vi "BioMapWriteCore.vi"(6 "conv. coeff.":sgl=655.0, 7 "Image in":dbl[][][](array[numeric]), 8 "error in":errorcluster, 9 "Y_img":i32, 10 "Image Params":T1={"File Header"={"Start Position"=[], "StepWidth"=[0.05, 0.05], "Dimension"=[], "SpecLength"=10000}, "mzCali."=[0.0, 1.0, 0.0], "m/z_Array"=[0.0, 1.0, 0.0], "SampleRate"=0.0, "TrigDelay"=0.0, "file refnum"=refnum, "file path"=path "", "PeakOI"=[], "Binning"={"Enable"=FALSE, "BinType"=enum."ByScreen", "BinWidth"=0.5, "Maximum"=0.0, "Minimum"=0.0}} {"SampleRate" items=["50MS/s"=50000000.0, "100MS/s"=100000000.0, "125MS/s"=125000000.0, "200MS/s"=200000000.0, "250MS/s"=250000000.0, "500MS/s"=500000000.0, "1GS/s"=1000000000.0, "1.6GS/s"=1600000000.0]}, 11 "data buffer in":refnum<queue>) -> (0 "error out":errorcluster, 2 "file refnum out":refnum<file>, 5 "Image out":dbl[][][](array[numeric]))   [LabVIEW 2013]
uses:
  BioMAPWriterCoreParams.ctl
  Files/BinaryHeader.ctl
  ControlDef/SampleRateSelector.ctl
  Binning/BinType.ctl
panel:
  out "#element":i32
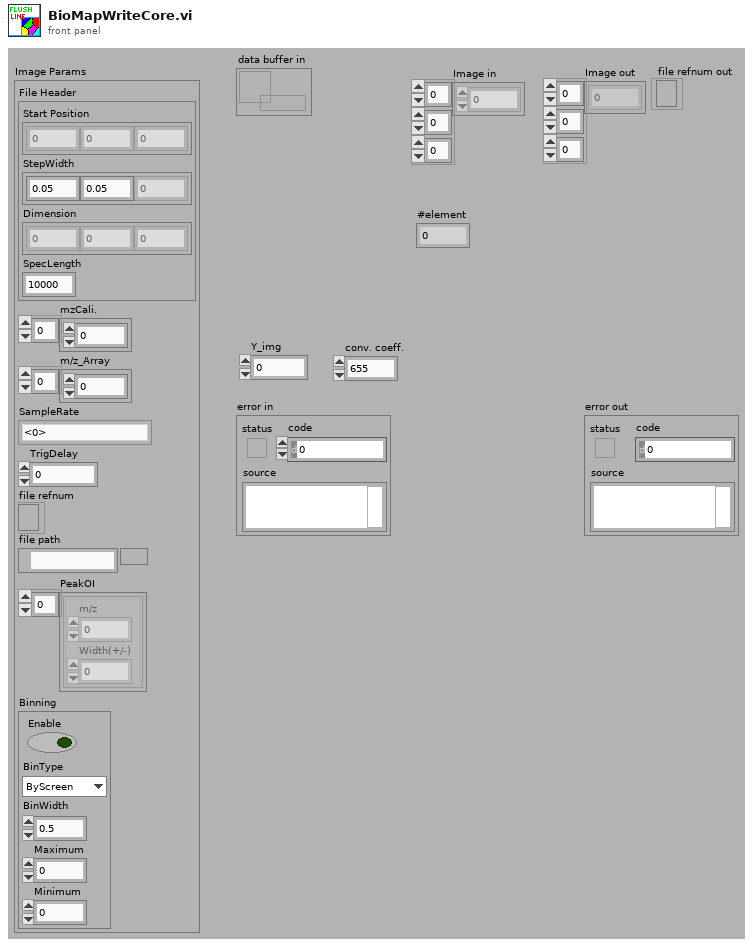
[diagram p1: front panel]
types:
  T1 = typedef "BioMAPWriterCoreParams.ctl" = cluster{"File Header":T2, "mzCali.":dbl[], "m/z_Array":dbl[], "SampleRate":T3, "TrigDelay":dbl, "file refnum":refnum<file>, "file path":path, "PeakOI":cluster{"m/z":dbl, "Width(+/-)":dbl}[], "Binning":cluster{"Enable":bool, "BinType":T4, "BinWidth":dbl, "Maximum":dbl, "Minimum":dbl}}
  T2 = typedef "BinaryHeader.ctl" = cluster{"Start Position":dbl[], "StepWidth":dbl[], "Dimension":i32[], "SpecLength":i32}
  T3 = typedef "SampleRateSelector.ctl" = dbl
  T4 = typedef "BinType.ctl" = enum16{"ByTime", "ByScreen", "ByMass", "ToUnitMass"}
  T5 = enum16{"big-endian, network order", "native, host order", "little-endian"}
  T6 = cluster{"Average":i32, "X (Img)":i32, "Y (Img)":i32, "Spectra":sgl[]}[]
  T7 = cluster{"Average":i32, "X (Img)":i32, "Y (Img)":i32, "Spectra":sgl[]}
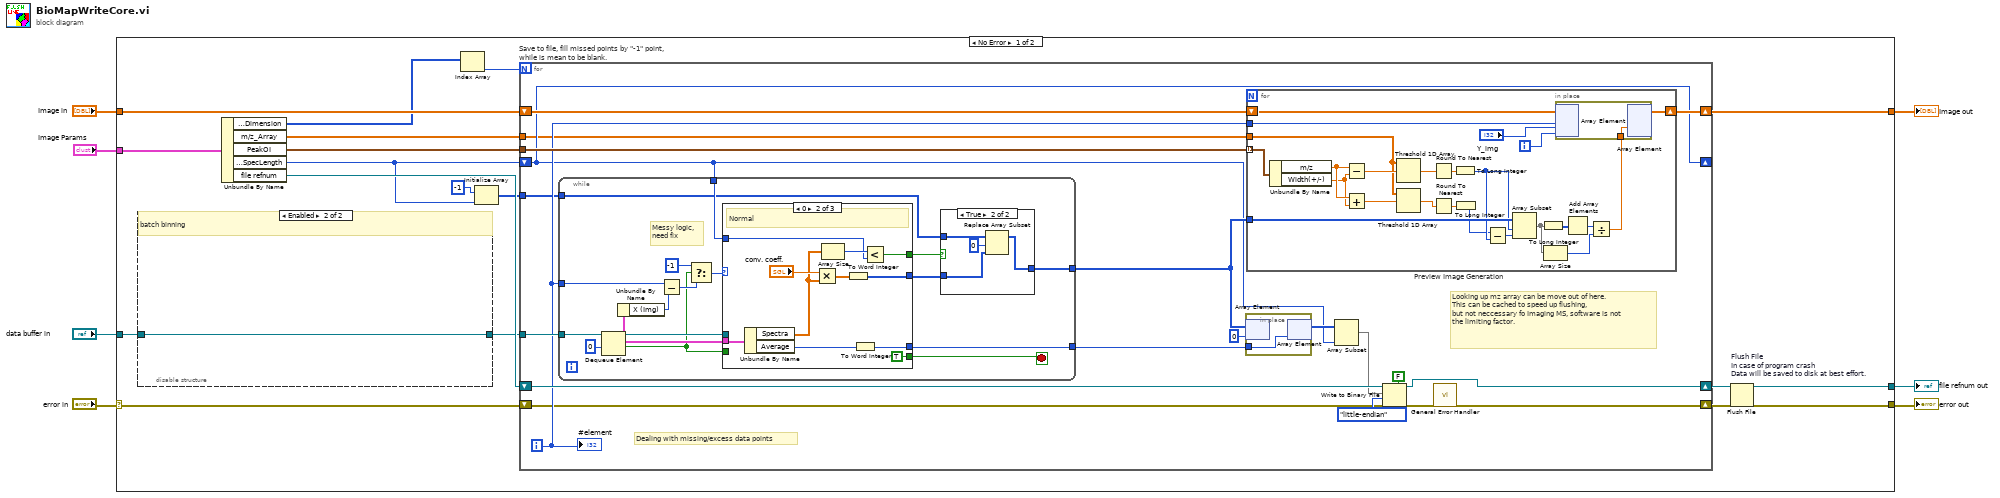
[diagram p0: block diagram]
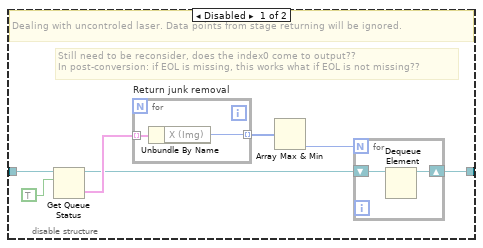
[diagram p2: hidden frame]
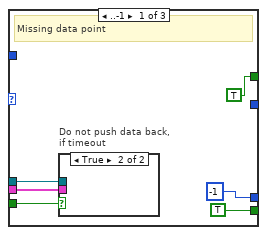
[diagram p4: hidden frame]
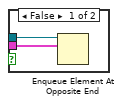
[diagram p5: hidden frame]
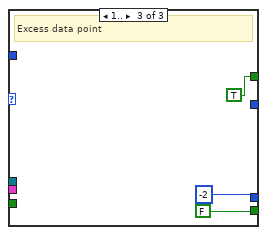
[diagram p6: hidden frame]
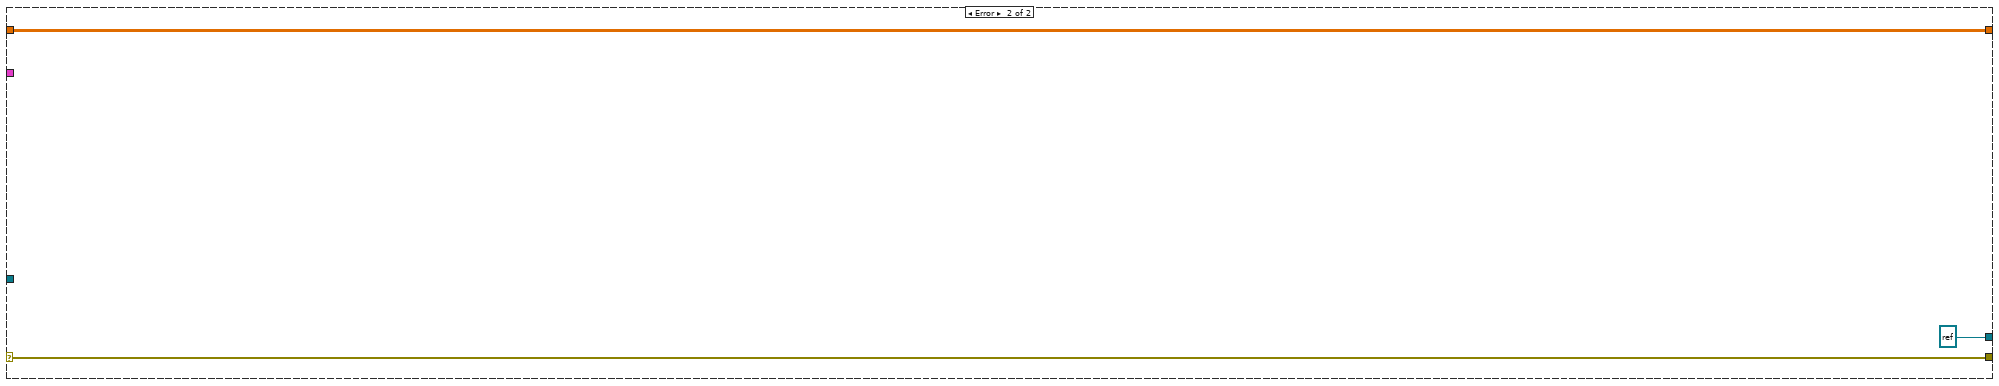
[diagram p7: hidden frame]
diagram:
  n1 = case shown="No Error" "error in" {
    selector: "error in" -> [w22 w130]
    tunnel: [w25 w128] -> w7
    tunnel: [w12 w130] -> w6
    tunnel: [w14 refnum<file> refnum ("file refnum")] -> w5
    tunnel: "Image in" -> [w23 w128]
    tunnel: "data buffer in" -> [w11 _]
    tunnel: "Image Params" -> [w9 _]
    frame No Error {
      n2 = disable-structure shown="Enabled" {
        disable-tunnel: w11 -> [w30 w37]
        disable-tunnel: [w28 w37] -> w17
        frame Disabled {
          # "Still need to be reconsider, does the index0 come to output??\nIn post-conversion: if EOL is missing, this works what if EOL is not missing??"
          # "Dealing with uncontroled laser. Data points from stage returning will be ignored."
          n3 = Get Queue Status(queue=w30, return elements? (F)=TRUE) -> (queue out=w29:refnum<queue>, elements=w32:T6)  [unwired: 1 in, 6 out]
          n4 = for "Return junk removal" {
            tunnel: w32 -> [w36] mode=indexing
            tunnel: [w35] -> w27 mode=indexing
            n5 = Unbundle By Name(w36) -> ("X (Img)"=w35:i32)
          }
          n6 = Array Max & Min(array=w27) -> (min index (indices)=w26:i32)  [unwired: 3 out]
          n7 = for {
            N: w26 -> [_]
            shift-right: [w33] -> w28
            shift-left: w29 -> [w34]
            n8 = Dequeue Element(queue=w34) -> (queue out=w33:refnum<queue>)  [unwired: 2 in, 3 out]
          }
        }
        frame Enabled {
          # "batch binning"
        }
      }
      n9 = Unbundle By Name(w9) -> ("File Header.Dimension"=w21:i32[], "m/z_Array"=w8:dbl[], "PeakOI"=w19:cluster{"m/z":dbl, "Width(+/-)":dbl}[], "File Header.SpecLength"=w10:i32, "file refnum"=w20:refnum<file>)
      n10 = Index Array(array=w21) -> (element=w18:i32)  [unwired: 1 in]
      n11 = Initialize Array(i16 -1 ("element"), w10) -> (w15:i16[])
      n12 = for "Save to file, fill missed points by \"-1\" point, while is mean to be blank." {
        N: w18 -> [_]
        shift-right: [w51] -> w13
        shift-left: w22 -> [w40]
        shift-right: [w54] -> w25
        shift-left: w23 -> [w53]
        tunnel: w17 -> [w57]
        shift-right: [w55] -> w24
        shift-left: w20 -> [w56]
        tunnel: w19 -> [w52]
        tunnel: w8 -> [w38]
        tunnel: w15 -> [w41]
        shift-right: [w39] -> _
        shift-left: w10 -> [w39]
        i -> [w42]
        # "Looking up mz array can be move out of here.\nThis can be cached to speed up flushing, \nbut not neccessary fo Imaging MS, software is not \nthe limiting factor."
        # "Dealing with missing/excess data points"
        n13 = while {
          tunnel: w57 -> [w74]
          tunnel: [w68] -> w44
          tunnel: w39 -> [w67]
          tunnel: [w62] -> w43
          tunnel: w42 -> [w63]
          tunnel: w41 -> [w60]
          stop <- w66 stop-if-true
          # "Messy logic,\nneed fix"
          n14 = Dequeue Element(queue=w74, timeout in ms (-1)=0) -> (queue out=w70:refnum<queue>, element=w69:T7, timed out?=w59:bool)  [unwired: 1 in, 1 out]
          n15 = Unbundle By Name(w69) -> ("X (Img)"=w72:i32)
          n16 = Subtract(x=w63, y=w72) -> (x-y=w71:i32)
          n17 = Select(t=-1, s=w59, f=w71) -> (s? t:f=w65:i32)
          n18 = case shown="0" w65 {
            tunnel: w70 -> [w82 _ _]
            tunnel: w69 -> [w81 w98 _]
            tunnel: [i16 -1 ("Average") w96 i16 -2 ("Average")] -> w68
            tunnel: w67 -> [_ w91 _]
            tunnel: [TRUE TRUE FALSE] -> w66
            tunnel: [_ w90 _] -> w61
            tunnel: [TRUE w89 TRUE] -> w58
            tunnel: w59 -> [w80 _ _]
            frame ..-1 {
              # "Missing data point"
              n19 = case "Do not push data back, \nif timeout" shown="True" w80 {
                tunnel: w82 -> [w87 _]
                tunnel: w81 -> [w86 _]
                frame False {
                  n20 = Enqueue Element At Opposite End(queue=w87, element=w86) -> ()  [unwired: 2 in, 3 out]
                }
                frame True {
                }
              }
            }
            frame 0 {
              # "Normal"
              n21 = Unbundle By Name(w98) -> ("Spectra"=w88:sgl[], "Average"=w95:i32)
              n22 = Multiply(x="conv. coeff.", y=w88) -> (x*y=w97:sgl[])
              n23 = Array Size(array=w88) -> (size(s)=w92:i32)
              n24 = To Word Integer(number=w97) -> (16bit integer=w90:i16[])
              n25 = To Word Integer(number=w95) -> (16bit integer=w96:i16)
              n26 = Less?(x=w92, y=w91) -> (x < y?=w89:bool)
            }
            frame 1.. {
              # "Excess data point"
            }
          }
          n27 = case shown="True" w58 {
            tunnel: [w75 w79] -> w62
            tunnel: w61 -> [w75 w77]
            tunnel: w60 -> [_ w78]
            frame False {
            }
            frame True {
              n28 = Replace Array Subset(array=w78, new element=w77, index=0) -> (w79:i16[])
            }
          }
        }
        n29 = in-place {
          in-place-border: w44 -> [w127]
          n30 = in-place-array #1(w43, 0) -> ()  [unwired: 1 out]
          n31 = in-place-array #1(w127) -> (w45:i16[])  [unwired: 1 out]
        }
        n32 = for "Preview Image Generation" {
          shift-right: [w112] -> w54
          shift-left: w53 -> [w119]
          tunnel: w52 -> [w125] mode=indexing
          tunnel: w43 -> [w118]
          tunnel: w38 -> [w121]
          tunnel: w42 -> [w105]
          i -> [w104]
          n33 = Unbundle By Name(w125) -> ("m/z"=w124:dbl, "Width(+/-)"=w123:dbl)
          n34 = Subtract(x=w124, y=w123) -> (x-y=w122:dbl)
          n35 = Add(x=w124, y=w123) -> (x+y=w120:dbl)
          n36 = Threshold 1D Array(2:w122, 3:w121) -> (0:w117:dbl)  [unwired: 1 in]
          n37 = Threshold 1D Array(2:w120, 3:w121) -> (0:w116:dbl)  [unwired: 1 in]
          n38 = Round To Nearest(number=w117) -> (nearest integer value=w113:dbl)
          n39 = Round To Nearest(number=w116) -> (nearest integer value=w114:dbl)
          n40 = To Long Integer(number=w113) -> (32bit integer=w111:i32)
          n41 = To Long Integer(number=w114) -> (32bit integer=w110:i32)
          n42 = Subtract(x=w110, y=w111) -> (x-y=w115:i32)
          n43 = Array Subset(array=w118, index=w111, length=w115) -> (w107:i16[])
          n44 = To Long Integer(number=w107) -> (32bit integer=w102:i32[])
          n45 = Array Size(array=w107) -> (size(s)=w108:i32)
          n46 = Add Array Elements(numeric array=w102) -> (sum=w109:i32)
          n47 = Divide(x=w109, y=w108) -> (x/y=w106:dbl)
          n48 = in-place {
            in-place-border: w106 -> [w126]
            n49 = in-place-array #2(w119, w105, "Y_img", w104) -> ()  [unwired: 1 out]
            n50 = in-place-array #2(w126) -> (w112:dbl[][][])  [unwired: 3 out]
          }
        }
        n51 = Array Subset(array=w45, length=w39) -> (w46:i16[])  [unwired: 1 in]
        n52 = Write to Binary File(file (use dialog)=w56, data=w46, error in=w40, 5:FALSE ("prepend array or string size? (T)"), 9:T5."little-endian" ("byte order (0:big-endian, network order)")) -> (refnum out=w55:refnum<file>, error out=w47:errorcluster)  [unwired: 1 in, 1 out]
        n53 = call <vilib>:"General Error Handler.vi"("error in (no error)"=w47) -> ("error out"=w51:errorcluster)  [unwired: 10 in, 4 out]
        "#element" <- w42
      }
      n54 = Flush File "Flush File\nIn case of program crash\nData will be saved to disk at best effort."(refnum=w24, error in=w13) -> (refnum out=w14:refnum<file>, error out=w12:errorcluster)
    }
    frame Error {
    }
  }
  "Image out" <- w7
  "error out" <- w6
  "file refnum out" <- w5
